vi "CP Plot Graph Formation.vi"(8 "CP A Tag AZ":string[](array[string]), 11 "CP Profile Table for plot":string[][](table) caption="CP Profile Table for Plot") -> (0 "layer":i32[](array[numeric]), 1 "Count Graph":cluster{i32[], i32[]}(graph) caption="ヒストグラムグラフ", 2 "Normalized Plot Graph":dbl[][](graph), 3 "Plot Graph":dbl[][](graph), 4 "Total Con and T":T3, 5 "R Con H":dbl[][](array[numeric]), 6 "Abs Plot Graph":dbl[][](graph), 7 "GAT":T1)   [LabVIEW 2018]
uses:
  <vilib>/Analysis/NI_AALPro.lvlib
  <vilib>/Analysis/NI_AALBase.lvlib
panel:
  out "エラー出力":errorcluster
  in  "エラー入力（エラーなし）":errorcluster
  out "x/y":dbl
  out "New MIN":dbl
  out "New MAX 2":dbl
  out "最大値 2":dbl
  out "Histogram 2":i32[](array[numeric]) caption="ヒストグラム"
  out "Histogram":i32[][](array[numeric])
  out "配列 2":dbl[][](array[numeric])
  out "配列":dbl[](array[numeric])
  out "GAF":T2
  out "Abs MIN 2":dbl
  out "Abs MAX 2":dbl
  out "Axis 2":dbl[](array[numeric])
  out "Abs MIN":dbl
  out "Abs MAX":dbl
  out "Axis":dbl[](array[numeric]) caption="軸" format="%0.2f"
  out "Abs Average":dbl[](array[numeric])
  out "T STD (%)":dbl[](array[numeric])
  out "T Average":dbl[](array[numeric])
  out "Time":dbl[](array[numeric])
  out "New bin":dbl
  out "New MAX":dbl
  out "STD (%)":dbl[](array[numeric])
  out "Average":dbl[](array[numeric])
  out "最大値":i32
  out "Relative Averaged Data":dbl[](array[numeric])
  out "AS IDX":i32[](array[numeric])
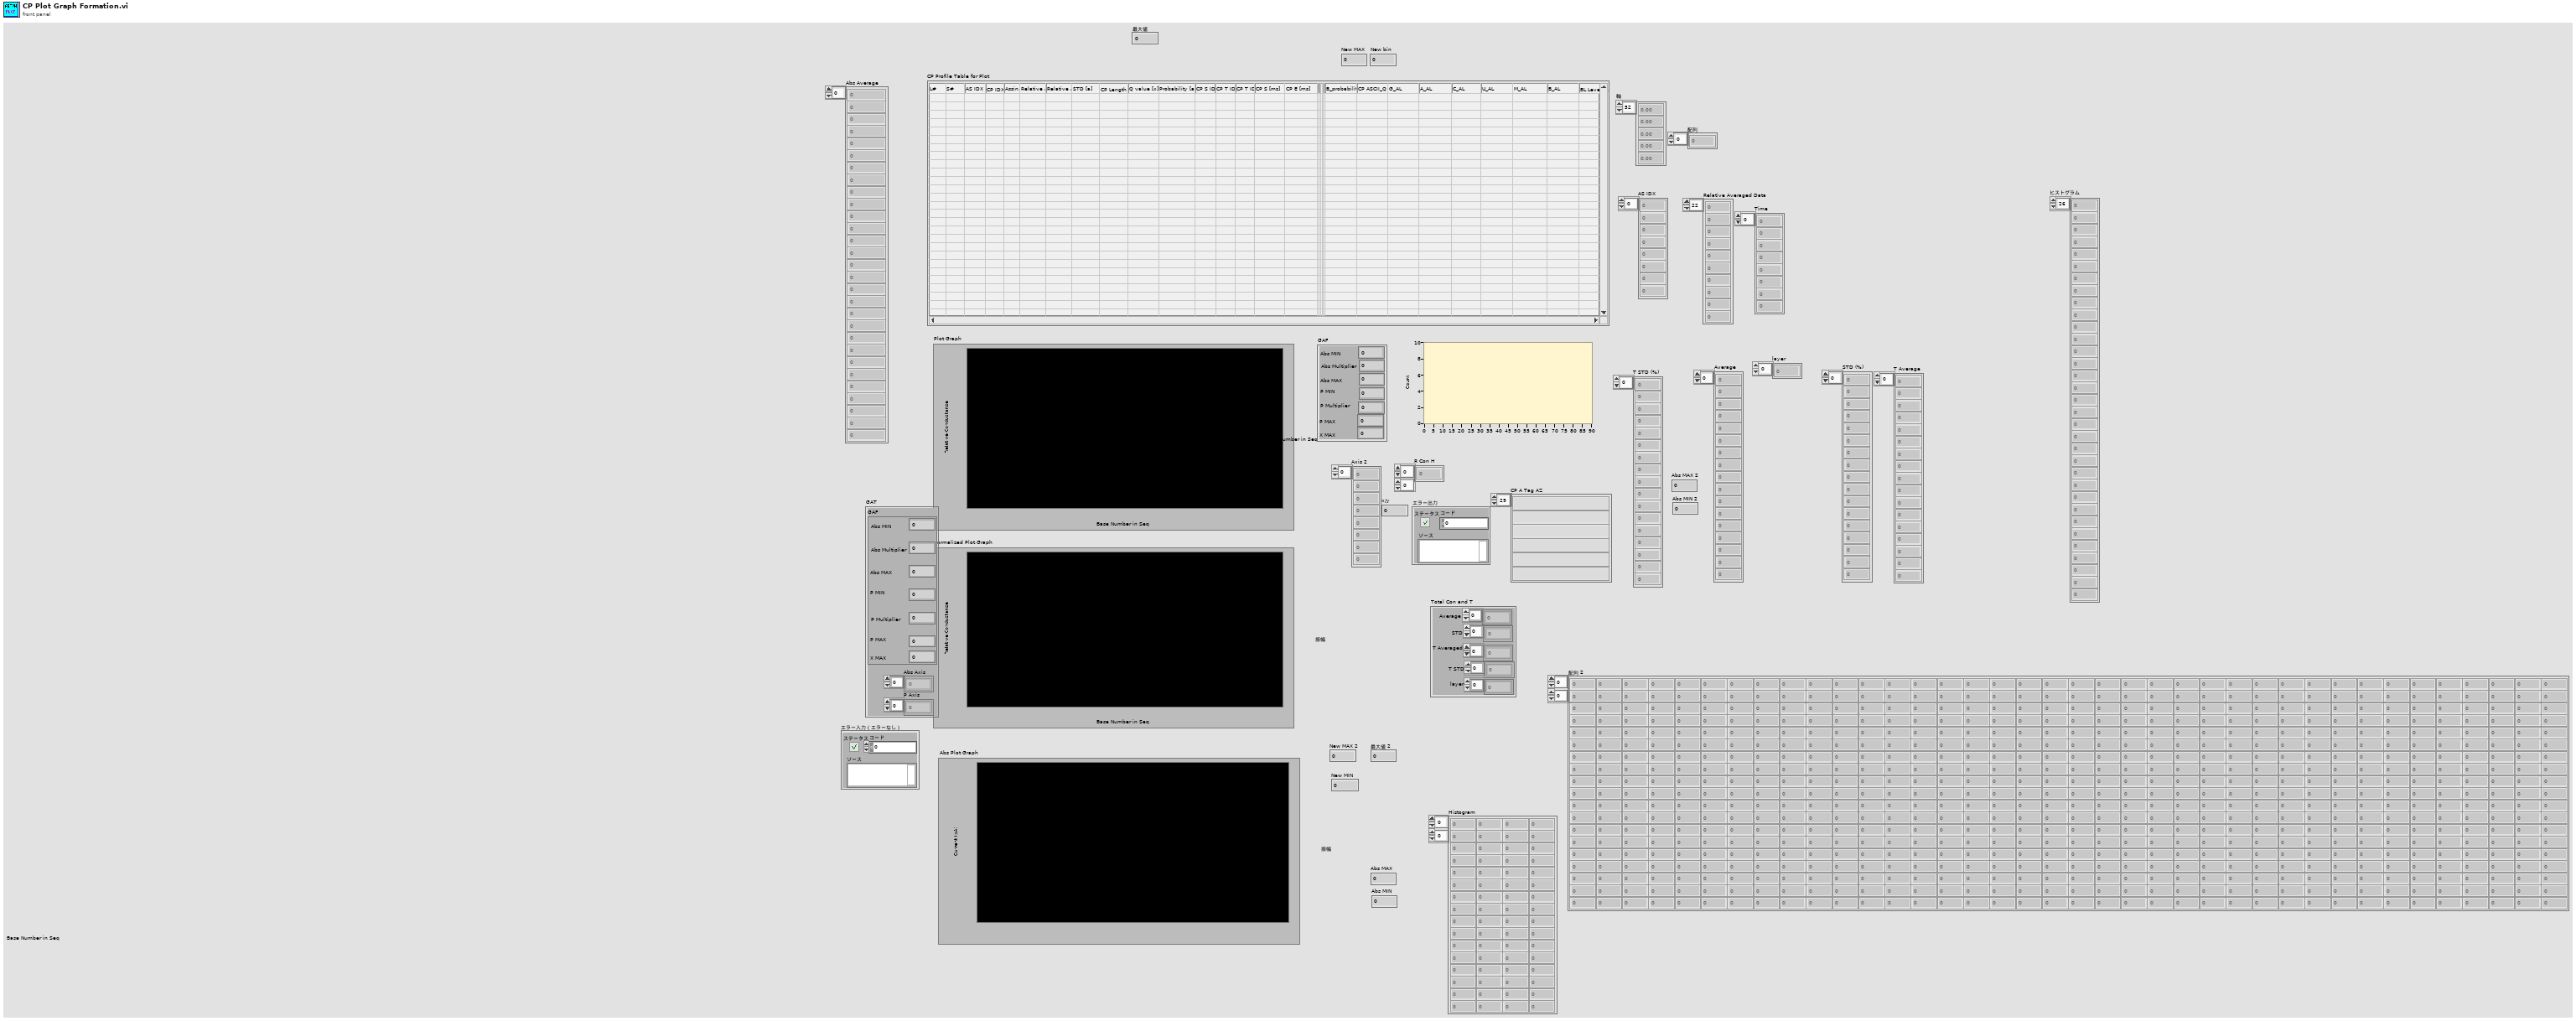
[diagram p1: front panel]
types:
  T1 = cluster{"GAF":cluster{"Abs MIN":dbl, "Abs Multiplier":dbl, "Abs MAX":dbl, "P MIN":dbl, "P Multiplier":dbl, "P MAX":dbl, "X MAX":dbl}, "Abs Axis":dbl[], "P Axis":dbl[]}
  T2 = cluster{"Abs MIN":dbl, "Abs Multiplier":dbl, "Abs MAX":dbl, "P MIN":dbl, "P Multiplier":dbl, "P MAX":dbl, "X MAX":dbl}
  T3 = cluster{"Average":dbl[], "STD":dbl[], "T Averaged":dbl[], "T STD":dbl[], "layer":i32[]}
  T4 = cluster{"Value":cluster{"Abs MIN":dbl, "Abs Multiplier":dbl, "Abs MAX":dbl, "P MIN":dbl, "P Multiplier":dbl, "P MAX":dbl, "X MAX":dbl}, "Axis":dbl[], "Axis":dbl[]}
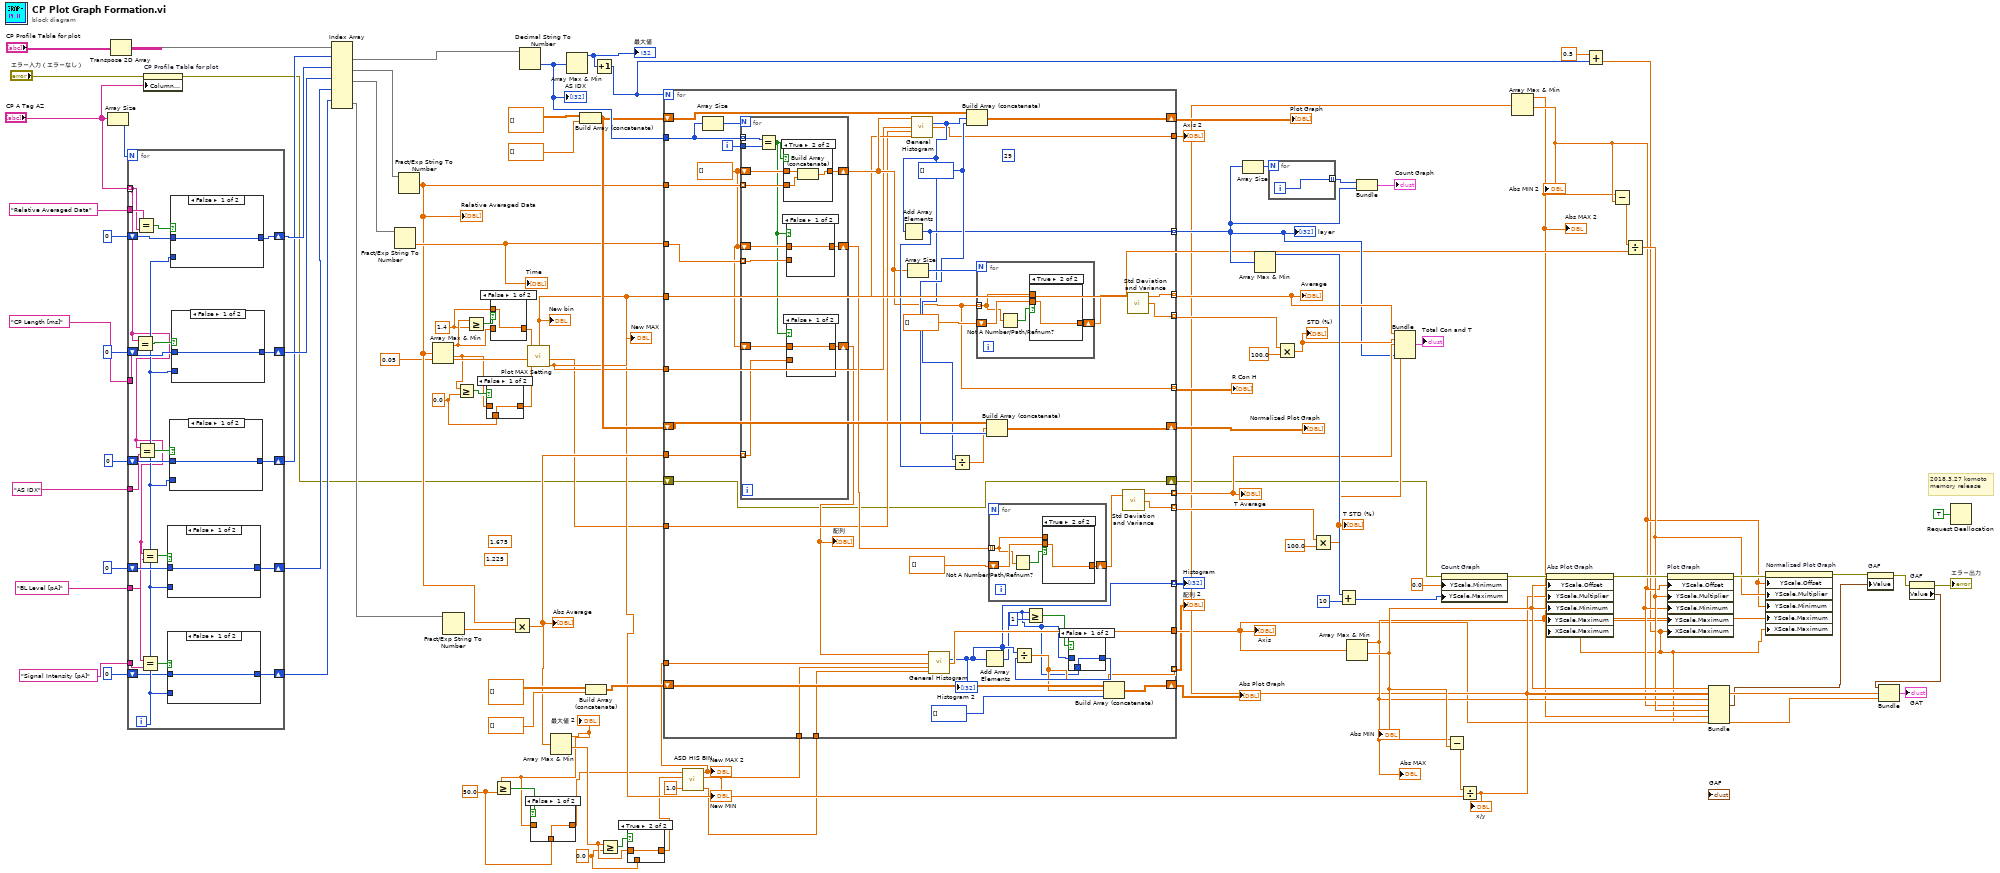
[diagram p0: block diagram]
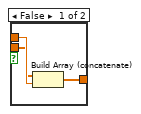
[diagram p12: hidden frame]
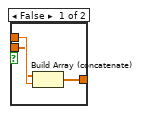
[diagram p13: hidden frame]
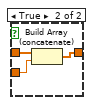
[diagram p14: hidden frame]
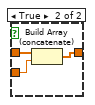
[diagram p15: hidden frame]
diagram:
  w10 = 50.0 ("最大値")
  w14 = 0.0 ("min")
  w20 = 0.0 ("min")
  (unwired) 1.225 ("max")
  (unwired) 1.675 ("max")
  w21 = 1.4 ("最大値")
  # "2018.3.27 komoto\nmemory release"
  n1 = Array Size(array="CP A Tag AZ") -> (size(s)=w87:i32)
  n2 = Transpose 2D Array(2D array="CP Profile Table for plot") -> (transposed array=w106:string[][])
  n3 = for {
    N: w87 -> [_]
    tunnel: "Relative Averaged Data" -> [w130]
    tunnel: "CP A Tag AZ" -> [w111] mode=indexing
    shift-right: [w128] -> w81
    shift-left: 0 -> [w127]
    tunnel: "CP Length [ms]" -> [w126]
    shift-right: [w124] -> w80
    shift-left: 0 -> [w123]
    shift-right: [w121] -> w66
    shift-left: 0 -> [w120]
    tunnel: "AS IDX" -> [w119]
    shift-right: [w117] -> w61
    shift-left: 0 -> [w118]
    shift-right: [w115] -> w60
    shift-left: 0 -> [w114]
    tunnel: "BL Level [pA]" -> [w110]
    tunnel: "Signal Intensity [pA]" -> [w109]
    i -> [w116]
    n4 = Equal?(x=w111, y=w126) -> (x = y?=w125:bool)
    n5 = Equal?(x=w130, y=w111) -> (x = y?=w129:bool)
    n6 = Equal?(x=w111, y=w119) -> (x = y?=w122:bool)
    n7 = Equal?(x=w111, y=w110) -> (x = y?=w113:bool)
    n8 = Equal?(x=w111, y=w109) -> (x = y?=w112:bool)
    n9 = case shown="False" w113 {
      tunnel: w116 -> [_ w134]
      tunnel: [w133 w134] -> w117
      tunnel: w118 -> [w133 _]
      frame False {
      }
      frame True {
      }
    }
    n10 = case shown="False" w112 {
      tunnel: w116 -> [_ w132]
      tunnel: [w131 w132] -> w115
      tunnel: w114 -> [w131 _]
      frame False {
      }
      frame True {
      }
    }
    n11 = case shown="False" w122 {
      tunnel: w116 -> [_ w136]
      tunnel: [w135 w136] -> w121
      tunnel: w120 -> [w135 _]
      frame False {
      }
      frame True {
      }
    }
    n12 = case shown="False" w129 {
      tunnel: w116 -> [_ w140]
      tunnel: [w139 w140] -> w128
      tunnel: w127 -> [w139 _]
      frame False {
      }
      frame True {
      }
    }
    n13 = case shown="False" w125 {
      tunnel: w116 -> [_ w138]
      tunnel: [w137 w138] -> w124
      tunnel: w123 -> [w137 _]
      frame False {
      }
      frame True {
      }
    }
  }
  n14 = property on="CP Profile Table for plot" class="Tbl (strict)"(error in="エラー入力（エラーなし）", "Column Headers[]"="CP A Tag AZ") -> (error out=w8:errorcluster)  [unwired: 1 in, 1 out]
  n15 = Index Array(array=w106, index (row) #1=w66, index (row) #2=w81, index (row) #3=w80, index (row) #4=w61, index (row) #5=w60) -> (element #1=w107:string[], element #2=w100:string[], element #3=w79:string[], element #5=w54:string[])  [unwired: 5 in, 1 out]
  n16 = Fract/Exp String To Number(string=w79) -> (number=w78:dbl[])  [unwired: 3 in, 1 out]
  "Time" <- w78
  n17 = Fract/Exp String To Number(string=w100) -> (number=w37:dbl[])  [unwired: 3 in, 1 out]
  "Relative Averaged Data" <- w37
  n18 = Array Max & Min(array=w37) -> (max value=w26:dbl, min value=w23:dbl)  [unwired: 2 out]
  n19 = Fract/Exp String To Number(string=w54) -> (number=w55:dbl[])  [unwired: 3 in, 1 out]
  n20 = Greater Or Equal?(x=w23, y=w20) -> (x >= y?=w24:bool)
  n21 = Greater Or Equal?(x=w26, y=w21) -> (x >= y?=w27:bool)
  n22 = case shown="False" w24 {
    tunnel: w23 -> [_ w142]
    tunnel: [w141 w142] -> w22
    tunnel: w20 -> [w141 _]
    frame False {
    }
    frame True {
    }
  }
  n23 = case shown="False" w27 {
    tunnel: w26 -> [_ w144]
    tunnel: [w143 w144] -> w25
    tunnel: w21 -> [w143 _]
    frame False {
    }
    frame True {
    }
  }
  n24 = Multiply(x=w37, y=w55) -> (x*y=w52:dbl[])
  "Abs Average" <- w52
  n25 = Decimal String To Number(string=w107) -> (number=w104:i32[])  [unwired: 2 in, 1 out]
  "AS IDX" <- w104
  n26 = call "Plot MAX Setting.vi"("min"=w22, "bin length"=0.05, "MAX"=w25) -> ("New MAX"=w88:dbl, "New MIN"=w35:dbl, "New bin"=w48:dbl)  [unwired: 6 in]
  "New MAX" <- w88
  "New bin" <- w48
  n27 = Array Max & Min(array=w52) -> (max value=w12:dbl, min value=w15:dbl)  [unwired: 2 out]
  "最大値 2" <- w12
  n28 = Greater Or Equal?(x=w12, y=w10) -> (x >= y?=w13:bool)
  n29 = case shown="False" w13 {
    tunnel: w12 -> [_ w146]
    tunnel: [w145 w146] -> w11
    tunnel: w10 -> [w145 _]
    frame False {
    }
    frame True {
    }
  }
  n30 = Array Max & Min(array=w104) -> (max value=w105:i32)  [unwired: 3 out]
  "最大値" <- w105
  n31 = Build Array (concatenate)(dbl[][] [] ("配列タイプ（2次元Dbl）"), dbl[] [] ("配列")) -> (w97:dbl[][])
  n32 = Build Array (concatenate)(dbl[][] [] ("配列タイプ（2次元Dbl）"), dbl[] [] ("配列")) -> (w57:dbl[][])
  n33 = Increment(x=w105) -> (x+1=w30:i32)
  n34 = Greater Or Equal?(x=w15, y=w14) -> (x >= y?=w17:bool)
  n35 = case shown="True" w17 {
    tunnel: w15 -> [_ w148]
    tunnel: [w147 w148] -> w16
    tunnel: w14 -> [w147 _]
    frame False {
    }
    frame True {
    }
  }
  n36 = call "ASD HIS BIN.vi"("bin length"=1.0, "min"=w16, "MAX"=w11) -> ("New bin"=w38:dbl, "New MIN"=w40:dbl, "New MAX"=w39:dbl)  [unwired: 6 in]
  "New MAX 2" <- w39
  "New MIN" <- w40
  n37 = for {
    N: w30 -> [_]
    tunnel: w37 -> [w190]
    tunnel: w104 -> [w192]
    shift-right: [w189] -> w102
    shift-left: w97 -> [w188]
    tunnel: [w180] -> w70 mode=indexing
    tunnel: [w187] -> w75 mode=indexing
    tunnel: [w186] -> w98 mode=indexing
    shift-right: [w177] -> w96
    shift-left: w97 -> [w182]
    tunnel: w88 -> [w163]
    tunnel: w48 -> [w164]
    tunnel: w78 -> [w176]
    tunnel: [w175] -> w73 mode=indexing
    tunnel: [w174] -> w76 mode=indexing
    tunnel: [w170] -> w69 mode=indexing
    shift-right: [w168] -> w56
    shift-left: w57 -> [w169]
    tunnel: w52 -> [w167]
    tunnel: w39 -> [w162]
    tunnel: w40 -> [w161]
    tunnel: [w160] -> w43
    tunnel: [w159] -> w44
    tunnel: w38 -> [w158]
    tunnel: w35 -> [w157]
    tunnel: [w152] -> w19 mode=indexing
    tunnel: [w151] -> w18 mode=indexing
    shift-right: [w149] -> w7
    shift-left: w8 -> [w149]
    i -> [w191]
    w181 = i32[] [] ("配列")
    (unwired) 29 ("# bins")
    w166 = dbl[] []
    n38 = Array Size(array=w192) -> (size(s)=w193:i32)
    n39 = for {
      N: w193 -> [_]
      tunnel: w192 -> [w223] mode=indexing
      tunnel: w191 -> [w222]
      tunnel: w190 -> [w221] mode=indexing
      shift-right: [w219] -> w170
      shift-left: w166 -> [w220]
      tunnel: w176 -> [w218] mode=indexing
      shift-right: [w217] -> w172
      shift-left: w166 -> [w216]
      tunnel: w167 -> [w215] mode=indexing
      shift-right: [w214] -> w153
      shift-left: w166 -> [w213]
      n40 = Equal?(x=w223, y=w222) -> (x = y?=w212:bool)
      n41 = case shown="True" w212 {
        tunnel: w221 -> [_ w235]
        tunnel: [w232 w234] -> w219
        tunnel: w220 -> [w232 w233]
        frame False {
        }
        frame True {
          n42 = Build Array (concatenate)(w233, w235) -> (w234:dbl[])
        }
      }
      n43 = case shown="False" w212 {
        tunnel: w218 -> [_ w231]
        tunnel: [w228 w230] -> w217
        tunnel: w216 -> [w228 w229]
        frame False {
        }
        frame True {
          n44 = Build Array (concatenate)(w229, w231) -> (w230:dbl[])
        }
      }
      n45 = case shown="False" w212 {
        tunnel: w215 -> [_ w227]
        tunnel: [w224 w226] -> w214
        tunnel: w213 -> [w224 w225]
        frame False {
        }
        frame True {
          n46 = Build Array (concatenate)(w225, w227) -> (w226:dbl[])
        }
      }
    }
    "配列" <- w153
    n47 = Array Size(array=w170) -> (size(s)=w185:i32)
    n48 = call <vilib>:"General Histogram.vi"("X"=w170, "max"=w163, "min"=w157, "# bins"=w164) -> ("Histogram"=w179:i32[], "Axis"=w159:dbl[])  [unwired: 7 in, 3 out]
    n49 = Add Array Elements(numeric array=w179) -> (sum=w180:i32)
    n50 = call <vilib>:"General Histogram.vi"("X"=w153, "max"=w162, "min"=w161, "# bins"=w158) -> ("Histogram"=w151:i32[], "Axis"=w160:dbl[])  [unwired: 7 in, 3 out]
    "Histogram 2" <- w151
    n51 = Divide(x=w179, y=w180) -> (x/y=w178:dbl[])
    n52 = Build Array (concatenate)(w188, w179, w181) -> (w189:dbl[][])
    n53 = for {
      N: w185 -> [_]
      tunnel: w170 -> [w205] mode=indexing
      shift-right: [w207] -> w183
      shift-left: dbl[] [] -> [w206]
      n54 = Not A Number/Path/Refnum?(number/path/refnum=w205) -> (NaN/Path/Refnum?=w204:bool)
      n55 = case shown="True" w204 {
        tunnel: w205 -> [w210 _]
        tunnel: [w209 w211] -> w207
        tunnel: w206 -> [w208 w211]
        frame False {
          n56 = Build Array (concatenate)(w208, w210) -> (w209:dbl[])
        }
        frame True {
        }
      }
    }
    n57 = Add Array Elements(numeric array=w151) -> (sum=w150:i32)
    n58 = Build Array (concatenate)(w182, w178, w181) -> (w177:dbl[][])
    n59 = for {
      tunnel: w172 -> [w197] mode=indexing
      shift-right: [w199] -> w171
      shift-left: dbl[] [] ("配列") -> [w198]
      n60 = Not A Number/Path/Refnum?(number/path/refnum=w197) -> (NaN/Path/Refnum?=w196:bool)
      n61 = case shown="True" w196 {
        tunnel: w197 -> [w202 _]
        tunnel: [w201 w203] -> w199
        tunnel: w198 -> [w200 w203]
        frame False {
          n62 = Build Array (concatenate)(w200, w202) -> (w201:dbl[])
        }
        frame True {
        }
      }
    }
    n63 = Greater Or Equal?(x=w150, y=1) -> (x >= y?=w156:bool)
    n64 = case shown="False" w156 {
      tunnel: w150 -> [_ w195]
      tunnel: [w194 w195] -> w154
      tunnel: w150 -> [w194 _]
      frame False {
      }
      frame True {
      }
    }
    n65 = Divide(x=w151, y=w154) -> (x/y=w152:dbl[])
    n66 = Build Array (concatenate)(w169, w152, i32[] [] ("配列")) -> (w168:dbl[][])
    n67 = call <vilib>:"Std Deviation and Variance.vi"("X"=w171) -> ("mean"=w175:dbl, "standard deviation"=w174:dbl)  [unwired: 1 in, 1 out]
    n68 = call <vilib>:"Std Deviation and Variance.vi"("X"=w183) -> ("mean"=w187:dbl, "standard deviation"=w186:dbl)  [unwired: 1 in, 1 out]
  }
  "Plot Graph" <- w102
  "layer" <- w70
  "Average" <- w75
  "Normalized Plot Graph" <- w96
  "T Average" <- w73
  "R Con H" <- w69
  "Abs Plot Graph" <- w56
  "Axis" <- w43
  "Axis 2" <- w44
  "配列 2" <- w19
  "Histogram" <- w18
  n69 = Array Size(array=w70) -> (size(s)=w95:i32)
  n70 = Array Max & Min(array=w70) -> (max value=w93:i32)  [unwired: 3 out]
  n71 = for {
    N: w95 -> [_]
    tunnel: [w236] -> w94 mode=indexing
    i -> [w236]
  }
  n72 = Multiply(x=w98, y=100.0) -> (x*y=w74:dbl[])
  "STD (%)" <- w74
  n73 = Multiply(x=w76, y=100.0) -> (x*y=w72:dbl[])
  "T STD (%)" <- w72
  n74 = Add(x=w93, y=10) -> (x+y=w89:i32)
  n75 = Array Max & Min(array=w43) -> (max value=w45:dbl, min value=w47:dbl)  [unwired: 2 out]
  "Abs MAX" <- w45
  "Abs MIN" <- w47
  n76 = Bundle(w94, w70) -> (→"Count Graph":cluster{i32[], i32[]})  [unwired: 1 in]
  n77 = Bundle(w75, w74, w73, w72, w70) -> (→"Total Con and T":cluster{dbl[], dbl[], dbl[], dbl[], i32[]})  [unwired: 1 in]
  n78 = property on="Count Graph" class="XYGraph (strict)"(error in=w7, "YScale.Minimum"=0.0 ("Yスケール.範囲:最小値"), "YScale.Maximum"=w89) -> (error out=w53:errorcluster)  [unwired: 1 in, 1 out]
  n79 = Subtract(x=w45, y=w47) -> (x-y=w51:dbl)
  n80 = Divide(x=w51, y=w48) -> (x/y=w46:dbl)
  "x/y" <- w46
  n81 = Array Max & Min(array=w44) -> (max value=w31:dbl, min value=w32:dbl)  [unwired: 2 out]
  "Abs MAX 2" <- w31
  "Abs MIN 2" <- w32
  n82 = Add(x=0.5, y=w30) -> (x+y=w28:dbl)
  n83 = property on="Abs Plot Graph" class="IntGraph (strict)"(error in=w53, "YScale.Offset"=w47, "YScale.Multiplier"=w46, "YScale.Minimum"=w47, "YScale.Maximum"=w45, "XScale.Maximum"=w28) -> (error out=w50:errorcluster)  [unwired: 1 in, 1 out]
  n84 = Subtract(x=w31, y=w32) -> (x-y=w49:dbl)
  n85 = Divide(x=w49, y=w48) -> (x/y=w33:dbl)
  n86 = property on="Plot Graph" class="IntGraph (strict)"(error in=w50, "YScale.Offset"=w32, "YScale.Multiplier"=w33, "YScale.Minimum"=w32, "YScale.Maximum"=w31, "XScale.Maximum"=w28) -> (error out=w34:errorcluster)  [unwired: 1 in, 1 out]
  n87 = Bundle(w47, w46, w45, w32, w33, w31, w28) -> (w5:cluster{dbl, dbl, dbl, dbl, dbl, dbl, dbl})  [unwired: 1 in]
  n88 = property on="Normalized Plot Graph" class="IntGraph (strict)"(error in=w34, "YScale.Offset"=w32, "YScale.Multiplier"=w33, "YScale.Minimum"=w32, "YScale.Maximum"=w31, "XScale.Maximum"=w28) -> (error out=w6:errorcluster)  [unwired: 1 in, 1 out]
  n89 = property on="GAF" class="Clust (strict)"(error in=w6, "Value"=w5) -> (error out=w4:errorcluster)  [unwired: 1 in, 1 out]
  n90 = property on="GAF" class="Clust (strict)"(error in=w4) -> (error out=→"エラー出力":errorcluster, "Value"=w2:T2)  [unwired: 1 in, 1 out]
  n91 = Bundle("Value"=w2, "Axis"=w44, "Axis"=w43) -> (→"GAT":T4)  [unwired: 1 in]
  n92 = Request Deallocation(TRUE ("フラグ")) -> ()
